vi "Create REST Client.vi"(4 "Default Headers ([JSON])":T1[](array[typedef])=[{"header"="Content-Type", "value"="application/json"}], 5 "REST Client in":refnum<class "REST Client.lvclass">, 6 "Verify Server(true)":bool=TRUE, 7 "Cookie File":path, 8 "error in (no error)":errorcluster, 9 "Authentication":cluster{"Username":string, "Password":string}, 10 "Escape URLs (true)":bool=TRUE, 11 "Base URL":string) -> (0 "error out":errorcluster, 3 "REST Client out":refnum<class "REST Client.lvclass">)   [LabVIEW 2020, in "REST Client.lvlib" / "REST Client.lvclass"]
doc: "The VI provides multiple arguments for defining how to create the JKI REST Client instance.\n\n<b>Base URL</b> specifies the base URL to be used for the HTTP requests.\n\n<b>Escape URLs</b> when true instruct the REST Client to escape all URLs before executing the requests. If you have already escaped the URLs, set this to false.\n\n<b>Authentication</b> allows setting the username and password for services that use HTTP authentication.\n\n<b>Verify Server</b> when true instructs the REST Client to validate the certificate of the server when HTTPS protocol is being used.\n\n<b>Default Headers</b> specifies an array of headers to be used with every requests. Defaults to application/json content type.\n\n<b>Cookie File</b> specifies a file path to be used for cookies."
uses:
  REST Client.lvclass
  HTTP Header.ctl
  <vilib>/NI/Advanced HTTP Client/Header--Combo Box.ctl
  REST Client.lvclass/REST Client.ctl
  http-client/http-client.lvclass
  <vilib>/NI/Advanced HTTP Client/Session.lvclass
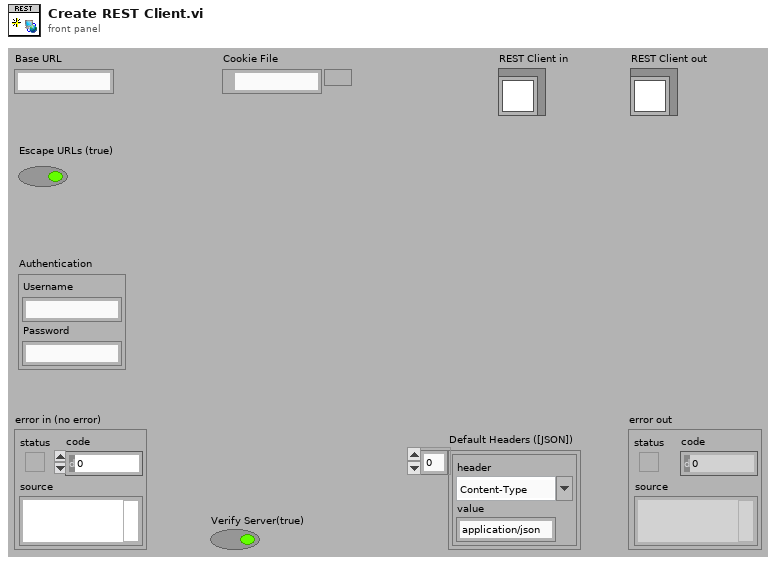
[diagram p1: front panel]
types:
  T1 = typedef "REST Client.lvlib/REST Client.lvclass/HTTP Header.ctl" = cluster{"header":T2, "value":string}
  T2 = typedef "lib_NI_Advanced HTTP Client.lvlib/Session.lvclass/Header--Combo Box.ctl" = string
  T3 = cluster{"http-client out":refnum<class "http-client.lvclass">, "Default Headers ([JSON])":T1[]}
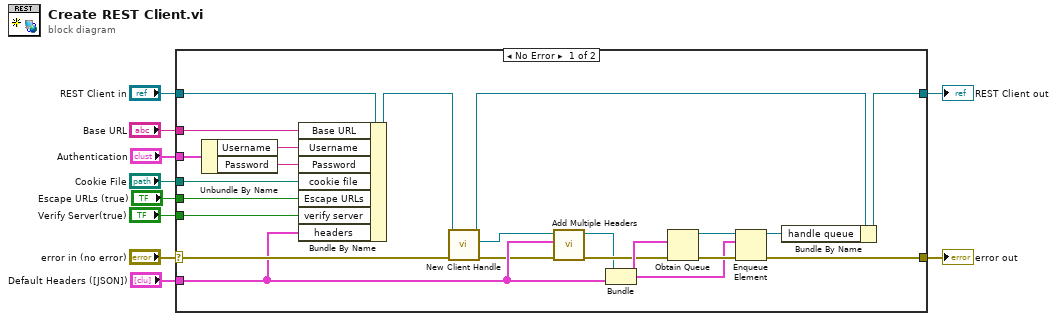
[diagram p0: block diagram]
diagram:
  n1 = case shown="No Error" "error in (no error)" {
    selector: "error in (no error)" -> [w31 w34]
    tunnel: [w26 w34] -> w9
    tunnel: [w12 w33] -> w7
    tunnel: "REST Client in" -> [w16 w33]
    tunnel: "Cookie File" -> [w30 _]
    tunnel: "Verify Server(true)" -> [w29 _]
    tunnel: "Default Headers ([JSON])" -> [w20 _]
    tunnel: "Authentication" -> [w24 _]
    tunnel: "Base URL" -> [w32 _]
    tunnel: "Escape URLs (true)" -> [w14 _]
    frame No Error {
      n2 = Unbundle By Name(w24) -> ("Username"=w23:string, "Password"=w22:string)
      n3 = Bundle By Name(cluster=w16, "Base URL"=w32, "Username"=w23, "Password"=w22, "cookie file"=w30, "Escape URLs"=w14, "verify server"=w29, "headers"=w20) -> (w15:refnum<class "REST Client.lvclass">)
      n4 = call "New Client Handle.vi"("error in (no error)"=w31, "REST Client in"=w15) -> ("error out"=w19:errorcluster, "http-client"=w21:refnum<class "http-client.lvclass">, "REST Client out"=w13:refnum<class "REST Client.lvclass">)  [unwired: 7 in]
      n5 = call "Add Multiple Headers.vi"("error in"=w19, "headers"=w20, "http-client in"=w21) -> ("error out"=w18:errorcluster, "http-client out"=w17:refnum<class "http-client.lvclass">)  [unwired: 7 in]
      n6 = Bundle("http-client out"=w17, "Default Headers ([JSON])"=w20) -> (w25:T3)  [unwired: 1 in]
      n7 = Obtain Queue(element data type=w25, error in (no error)=w18) -> (queue out=w28:refnum<queue>, error out=w27:errorcluster)  [unwired: 3 in, 1 out]
      n8 = Enqueue Element(queue=w28, element=w25, error in (no error)=w27) -> (queue out=w11:refnum<queue>, error out=w26:errorcluster)  [unwired: 1 in, 1 out]
      n9 = Bundle By Name(cluster=w13, "handle queue"=w11) -> (w12:refnum<class "REST Client.lvclass">)
    }
    frame Error {
    }
  }
  "error out" <- w9
  "REST Client out" <- w7
